vi "Format VI Info Column.vi"(8 "error in (no error)":errorcluster {"code" format="Error %.0f"}, 9 "Column":T9=enum."FP", 10 "VI Info":T1, 11 "VIDoc Printer - Confluence In":refnum<class "VIDoc Printer - Confluence.lvclass">) -> (0 "error out":errorcluster {"code" format="Error %.0f"}, 1 "Header":string, 2 "Cell Text":string, 3 "VIDoc Printer - Confluence Out":refnum<class "VIDoc Printer - Confluence.lvclass">, 4 "Viable Value?":bool, 5 "Pixel Width":i16=275)   [LabVIEW 2023, in "VIDoc Printer - Confluence.lvlib" / "VIDoc Printer - Confluence.lvclass"]
uses:
  VIDoc Printer - Confluence.lvclass
  C:/Program Files/National Instruments/LabVIEW 2023/vi.lib/DMC/VIDoc/Framework/Printer/VIDoc Printer.lvclass
  Confluence Printer Settings/VI Info Column.ctl
  <vilib>/DMC/VIDoc/Framework/Parsing/TypeDefs/Method Spec Cluster.ctl
  <vilib>/DMC/VIDoc/Framework/Parsing/TypeDefs/VI Type Extended Enum.ctl
  <vilib>/picture/picture.llb/imagedata.ctl
  <vilib>/DMC/VIDoc/Framework/Parsing/TypeDefs/Class Dispatch Type Enum.ctl
  <vilib>/DMC/VIDoc/Framework/Parsing/TypeDefs/Controls Info Cluster.ctl
  <vilib>/Utility/miscctls.llb/LVKeyTypeDef.ctl
  <vilib>/Utility/miscctls.llb/LVPointTypeDef.ctl
  <vilib>/DMC/VIDoc/Framework/Parsing/SubVIs/Structure Reporter/Tree Cluster.ctl
  Types/VI Info Image Types.ctl
  <vilib>/DMC/VIDoc/Framework/Printer/VIDoc Printer.lvclass/VIDoc Printer.ctl
  <vilib>/DMC/VIDoc/Framework/Printer/Accessors/Get Formatting Settings - Bookmark Options.vi
  <vilib>/DMC/VIDoc/Framework/Printer/Accessors/Get Formatting Settings.vi
  Accessors/Get Current Page Title.vi
  <userlib>/_PetranWay/LabVIEW Confluence API/Source/Confluence/HTML/Add Link to Text/Add URL to Text.vi
  VIDoc Printer - Confluence.lvclass/VIDoc Printer - Confluence.ctl
  <vilib>/DMC/VIDoc/Framework/Printer/VIDoc Printer.lvclass
  Confluence Formatting/Confluence Formatting.lvlib
  <userlib>/_PetranWay/LabVIEW Confluence API/Source/PetranWay_Confluence API.lvlib
  Confluence Printer Settings/VIDoc Settings - Confluence.lvclass
  <vilib>/DMC/VIDoc/Framework/Parsing/VIDoc Parsing.lvlib
  <vilib>/DMC/VIDoc/Framework/Parsing/SubVIs/Structure Reporter/Structure Reporter.lvlib
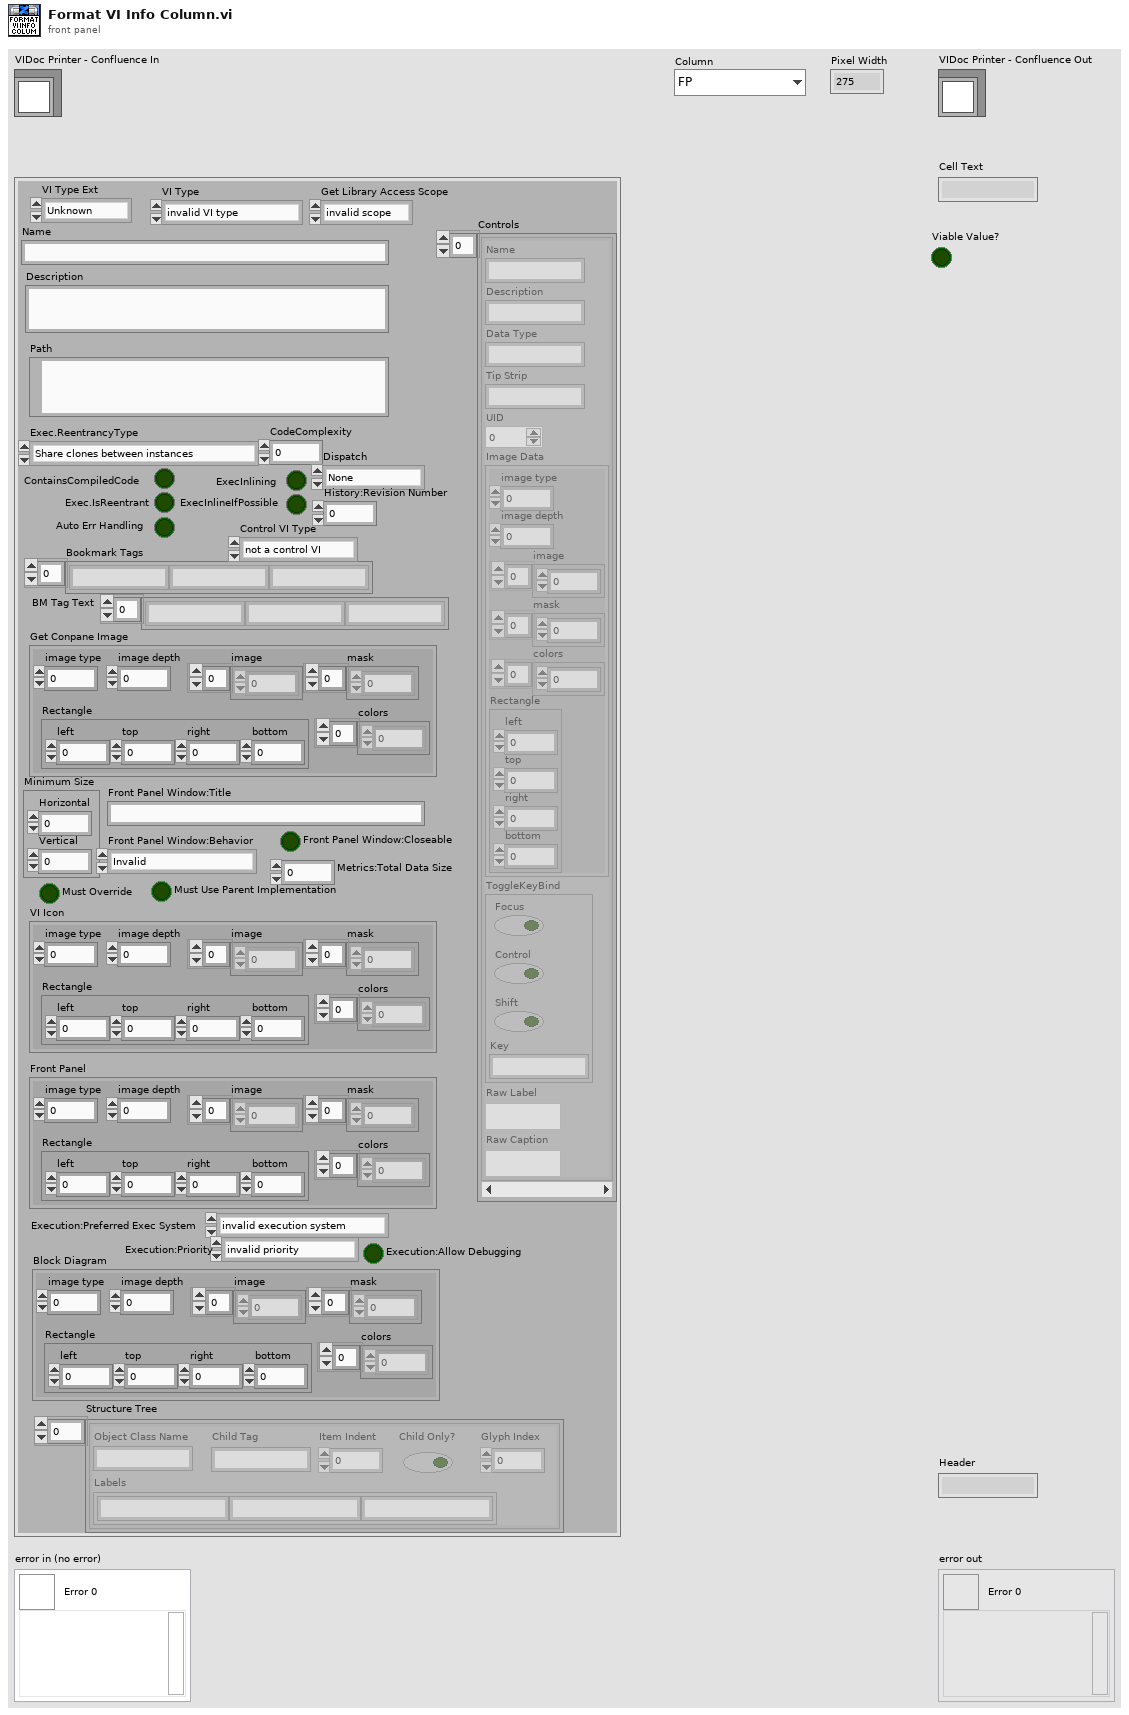
[diagram p1: front panel]
types:
  T1 = typedef "VIDoc Parsing.lvlib/Method Spec Cluster.ctl" = cluster{"VI Type Ext":T2, "Name":string, "Path":path, "Get Conpane Image":T3, "Description":string, "Get Library Access Scope":enum32{"invalid scope", "public", "private", "protected", "community"}, "Dispatch":T4, "ContainsCompiledCode":bool, "Exec.IsReentrant":bool, "Exec.ReentrancyType":enum16{"Share clones between instances", "Preallocate clone for each instance"}, "ExecInlining":bool, "ExecInlineIfPossible":bool, "Auto Err Handling":bool, "CodeComplexity":sgl, "Bookmark Tags":string[], "Control VI Type":enum32{"not a control VI", "control", "typedef", "strict typedef"}, "Controls":T5[], "VI Type":enum32{"invalid VI type", "Standard VI", "Control VI", "Global VI", "Polymorphic VI", "Configuration VI", "SubSystem", "Facade VI", "Method VI", "Statechart Diagram VI"}, "Minimum Size":T7, "Front Panel Window:Title":string, "Front Panel Window:Behavior":enum32{"Invalid", "Default", "Floating", "Floating/Auto-Hide", "Modal"}, "Front Panel Window:Closeable":bool, "Must Override":bool, "Must Use Parent Implementation":bool, "VI Icon":T3, "Front Panel":T3, "History:Revision Number":u32, "Metrics:Total Data Size":u32, "Execution:Allow Debugging":bool, "Execution:Preferred Exec System":enum32{"invalid execution system", "user interface", "standard", "instrument i/o", "data acquisition", "other 1", "other 2", "same as caller"}, "Execution:Priority":enum32{"invalid priority", "background priority", "normal priority", "above normal priority", "high priority", "time critical priority", "subroutine"}, "BM Tag Text":string[], "Block Diagram":T3, "Structure Tree":T8[]}
  T2 = typedef "VIDoc Parsing.lvlib/VI Type Extended Enum.ctl" = enum16{"Unknown", "Class Method", "Class Accessor Get", "Class Accessor Set", "Class Control", "Library Method", "Library Control", "VI", "Control"}
  T3 = typedef "imagedata.ctl" = cluster{"image type":i32, "image depth":i32, "image":u8[], "mask":u8[], "colors":u32[], "Rectangle":cluster{"left":i16, "top":i16, "right":i16, "bottom":i16}}
  T4 = typedef "VIDoc Parsing.lvlib/Class Dispatch Type Enum.ctl" = enum16{"None", "Static", "Dynamic"}
  T5 = typedef "VIDoc Parsing.lvlib/Controls Info Cluster.ctl" = cluster{"Name":string, "Description":string, "Data Type":string, "Tip Strip":string, "UID":i32, "Image Data":T3, "ToggleKeyBind":T6, "Raw Label":string, "Raw Caption":string}
  T6 = typedef "LVKeyTypeDef.ctl" = cluster{"Focus":bool, "Control":bool, "Shift":bool, "Key":string}
  T7 = typedef "LVPointTypeDef.ctl" = cluster{"Horizontal":i16, "Vertical":i16}
  T8 = typedef "VIDoc Parsing.lvlib/Structure Reporter.lvlib/Tree Cluster.ctl" = cluster{"Object Class Name":string, "Labels":string[], "Child Tag":string, "Item Indent":i32, "Child Only?":bool, "Glyph Index":i32}
  T9 = typedef "VIDoc Printer - Confluence.lvlib/VIDoc Settings - Confluence.lvclass/VI Info Column.ctl" = enum16{"Name", "Conpane", "BD", "FP", "VI Icon", "Description", "Reentrant", "Inline", "Auto Error", "Compiled", "Code Complexity", "Data Size", "Debug", "Priority", "Rev", "Minimum Size", "Title", "FP Behavior", "FP Closeable", "Author", "Commit Hash", "Last Change", "Branch", "Scope", "Type", "Dispatch", "Must Override", "Must Use Parent", "Structure Tree"}
  T10 = typedef "VIDoc Printer - Confluence.lvlib/VIDoc Printer - Confluence.lvclass/VI Info Image Types.ctl" = enum16{"Conpane", "FP", "BD", "Icon"}
  T11 = typedef "VIDoc Printer.lvlib/Printer Settings.lvclass/Bookmark Options.ctl" = cluster{"Bookmarks as New Line in VI Descriptions":bool, "Unique Bookmark Tags Only":bool, "Include Tag and Text":bool}
  T12 = enum16{"Share clones between instances", "Preallocate clone for each instance"}
  T13 = typedef "VIDoc Printer.lvlib/Printer Settings.lvclass/Formatting Options.ctl" = cluster{"Background":cluster{"Public Scope":T14, "Protected Scope":T14, "Community Scope":T14, "Private Scope":T14, "Unknown Scope":T14, "Auto Error Handling":T14, "Inline":T14, "Separate CC":T14, "Execution Priority Normal":T14, "Reentrancy Non-RE":T14}, "Bookmark Options":T11}
  T14 = typedef "VIDoc Printer.lvlib/Printer Settings.lvclass/Background Formatting Cluster.ctl" = cluster{"Option":bool, "Color":u32, "Operator":bool}
  T15 = enum32{"invalid priority", "background priority", "normal priority", "above normal priority", "high priority", "time critical priority", "subroutine"}
  T16 = enum32{"Invalid", "Default", "Floating", "Floating/Auto-Hide", "Modal"}
  T17 = cluster{"Timestamp":timestamp, "Commit Hash":string, "Author Name":string, "Branch":string, "Commit Hash URL":string}
  T18 = enum32{"invalid scope", "public", "private", "protected", "community"}
  T19 = enum32{"not a control VI", "control", "typedef", "strict typedef"}
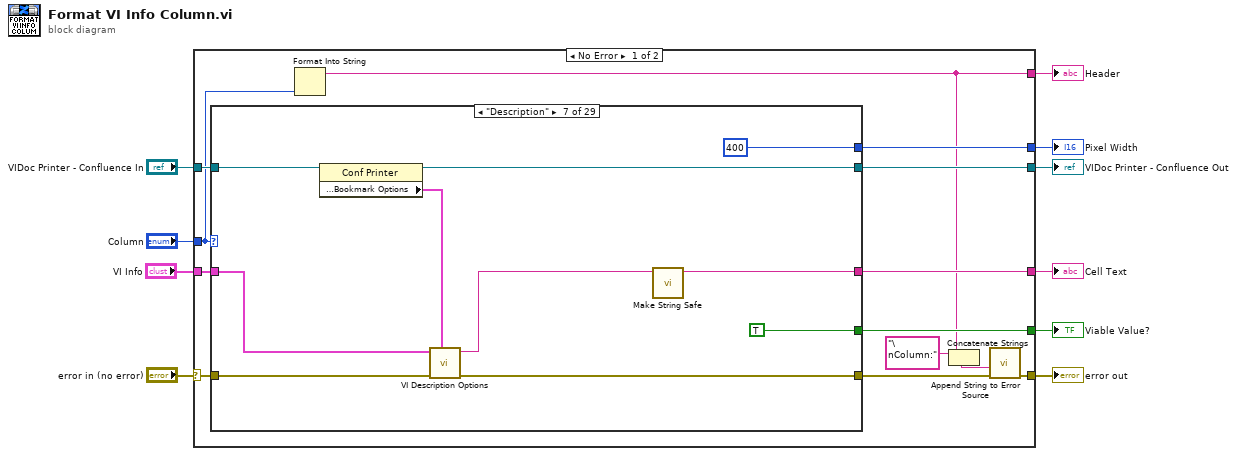
[diagram p0: block diagram]
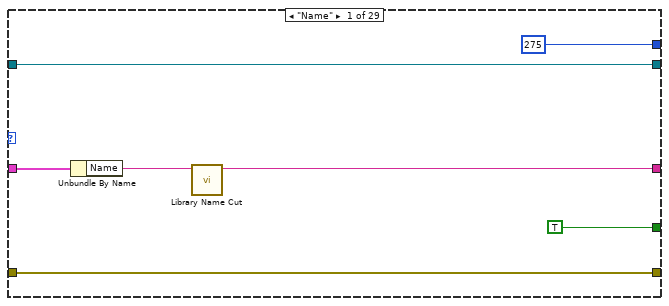
[diagram p2: hidden frame]
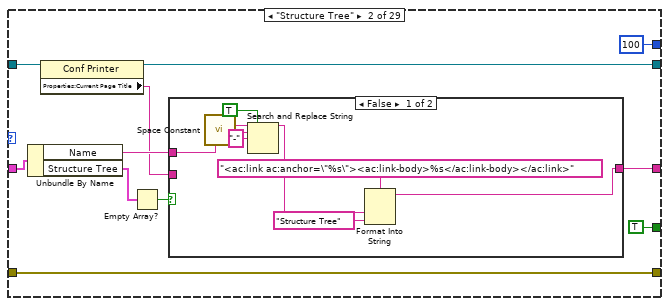
[diagram p3: hidden frame]
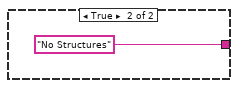
[diagram p4: hidden frame]
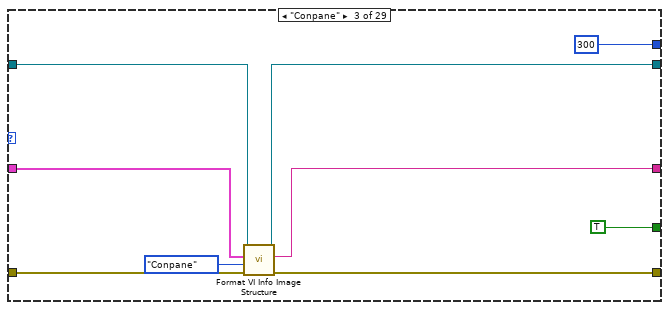
[diagram p5: hidden frame]
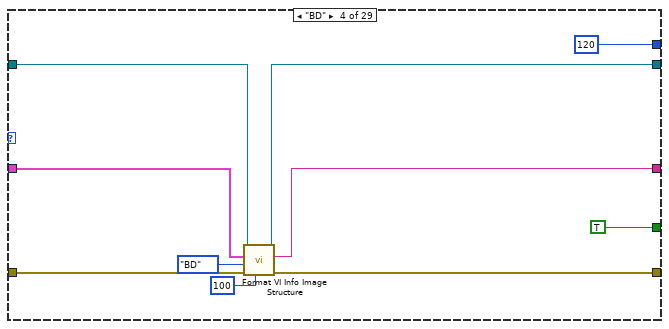
[diagram p6: hidden frame]
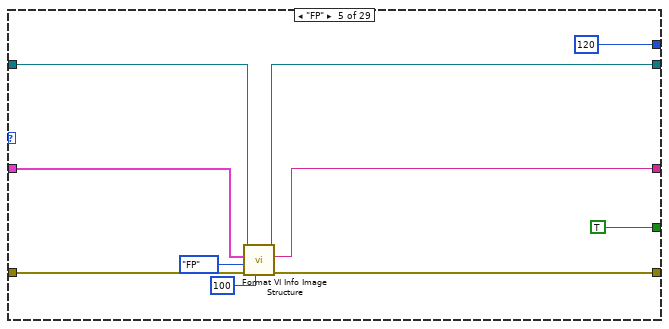
[diagram p7: hidden frame]
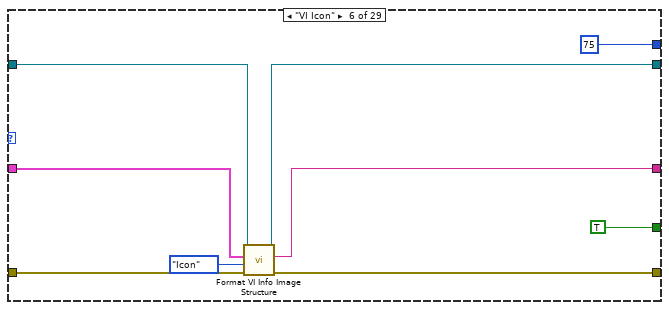
[diagram p8: hidden frame]
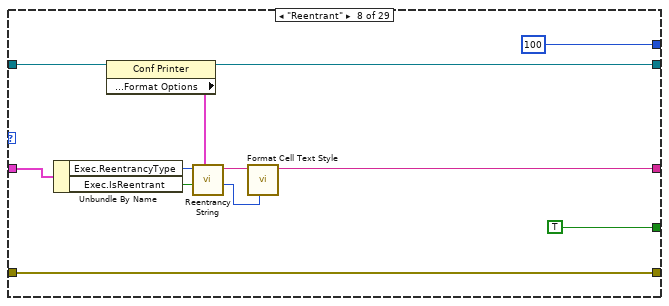
[diagram p9: hidden frame]
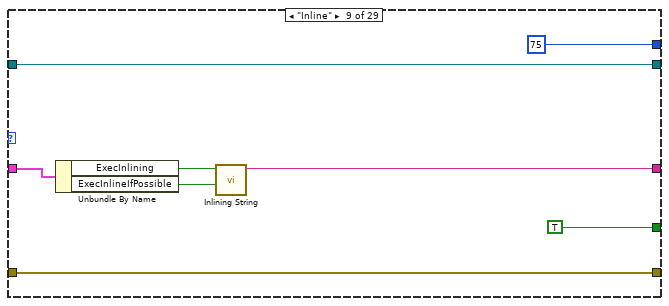
[diagram p10: hidden frame]
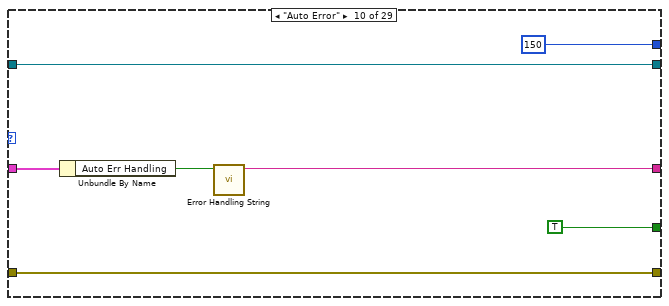
[diagram p11: hidden frame]
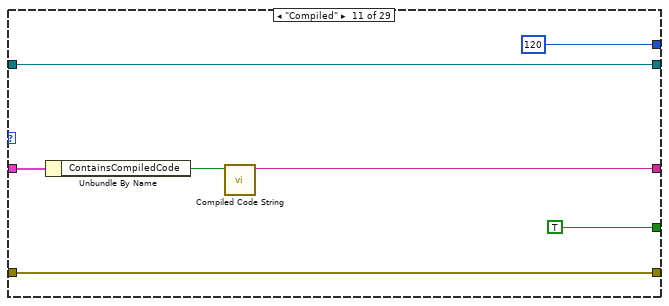
[diagram p12: hidden frame]
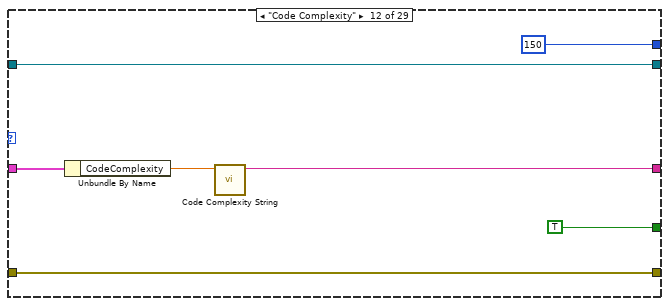
[diagram p13: hidden frame]
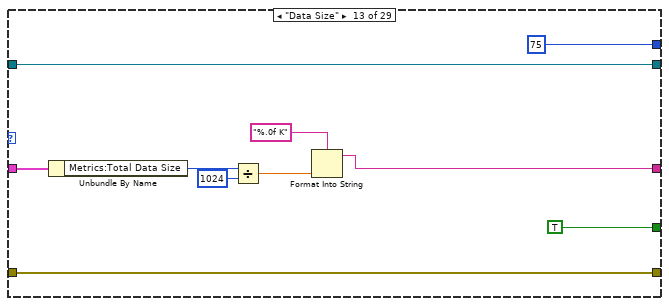
[diagram p14: hidden frame]
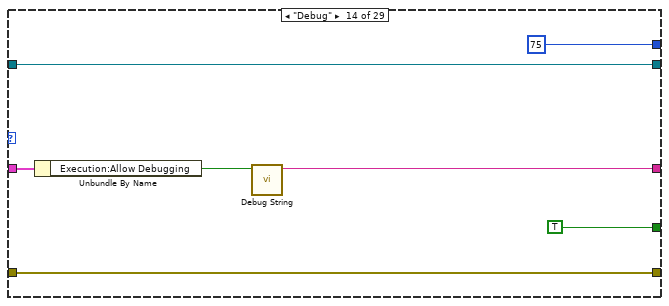
[diagram p15: hidden frame]
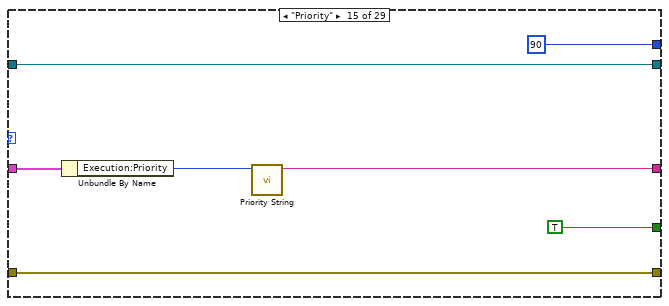
[diagram p16: hidden frame]
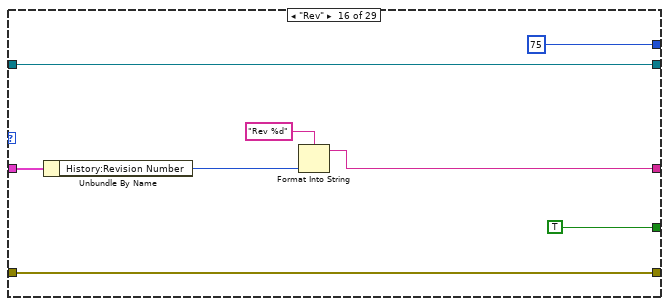
[diagram p17: hidden frame]
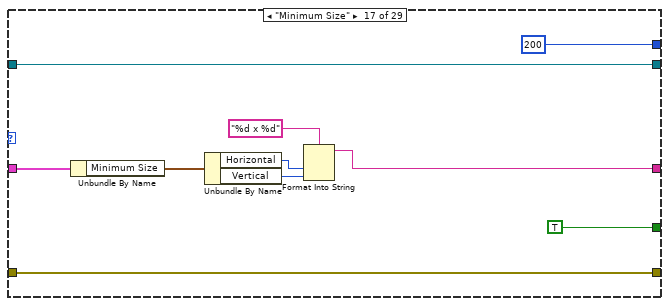
[diagram p18: hidden frame]
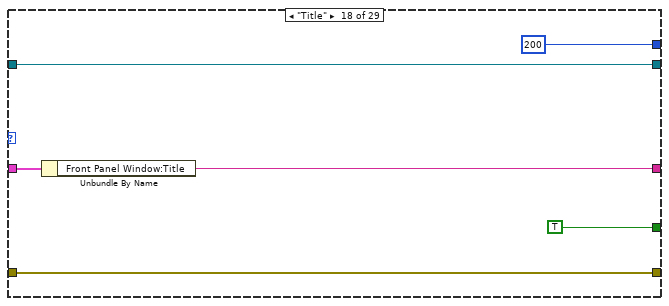
[diagram p19: hidden frame]
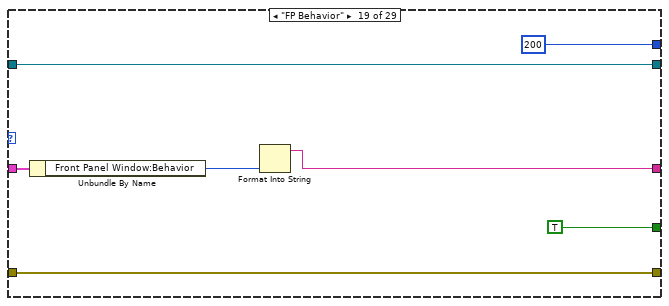
[diagram p20: hidden frame]
diagram:
  n1 = case shown="No Error" "error in (no error)" {
    selector: "error in (no error)" -> [w22 w293]
    tunnel: [w14 w293] -> w9
    tunnel: [w21 w292] -> w7
    tunnel: "VIDoc Printer - Confluence In" -> [w20 w292]
    tunnel: "Column" -> [w17 _]
    tunnel: "VI Info" -> [w19 _]
    tunnel: [w18 _] -> w4
    tunnel: [w12 _] -> w3
    tunnel: [w16 _] -> w2
    tunnel: [w15 FALSE ("File Change Info Available?")] -> w1
    frame No Error {
      n2 = case shown="\"Description\"" w17 {
        tunnel: [w30 w40 w55 w65 w75 w84 w91 w104 w115 w122 w129 w136 w146 w153 w160 w168 w178 w184 w191 w200 w211 w214 w243 w253 w262 w269 w273 w280 w287] -> w23
        tunnel: w22 -> [w30 w40 w58 w68 w78 w87 w96 w104 w115 w122 w129 w136 w146 w153 w160 w168 w178 w184 w191 w200 w210 w224 w242 w252 w262 w269 w273 w280 w287]
        tunnel: [w29 w32 w56 w66 w76 w85 w95 w108 w117 w124 w131 w138 w148 w155 w162 w170 w180 w186 w193 w202 w209 w223 w241 w251 w261 w268 w275 w282 w289] -> w21
        tunnel: w20 -> [w29 w41 w57 w67 w77 w86 w97 w109 w117 w124 w131 w138 w148 w155 w162 w170 w180 w186 w193 w202 w208 w222 w240 w250 w261 w268 w275 w282 w289]
        tunnel: w19 -> [w28 w39 w52 w62 w72 w81 w93 w107 w116 w123 w130 w137 w147 w154 w161 w169 w179 w185 w192 w201 w212 w225 w244 w254 w260 w267 w274 w281 w288]
        tunnel: [w25 w35 w54 w64 w74 w83 w89 w100 w112 w120 w127 w134 w141 w151 w158 w165 w173 w183 w189 w196 w205 w215 w235 w247 w256 w263 w270 w277 w284] -> w18
        tunnel: [i16 275 ("Pixel Width") i16 100 ("Pixel Width") i16 300 ("Pixel Width") i16 120 ("Pixel Width") i16 120 ("Pixel Width") i16 75 ("Pixel Width") i16 400 ("Pixel Width") i16 100 ("Pixel Width") i16 75 ("Pixel Width") i16 150 ("Pixel Width") i16 120 ("Pixel Width") i16 150 ("Pixel Width") i16 75 ("Pixel Width") i16 75 ("Pixel Width") i16 90 ("Pixel Width") i16 75 ("Pixel Width") i16 200 ("Pixel Width") i16 200 ("Pixel Width") i16 200 ("Pixel Width") i16 120 ("Pixel Width") i16 120 ("Pixel Width") i16 120 ("Pixel Width") i16 200 ("Pixel Width") i16 200 ("Pixel Width") i16 100 ("Pixel Width") i16 300 ("Pixel Width") i16 90 ("Pixel Width") i16 90 ("Pixel Width") i16 90 ("Pixel Width")] -> w16
        tunnel: [TRUE ("File Change Info Available?") TRUE ("File Change Info Available?") TRUE ("File Change Info Available?") TRUE ("File Change Info Available?") TRUE ("File Change Info Available?") TRUE ("File Change Info Available?") TRUE ("File Change Info Available?") TRUE ("File Change Info Available?") TRUE ("File Change Info Available?") TRUE ("File Change Info Available?") TRUE ("File Change Info Available?") TRUE ("File Change Info Available?") TRUE ("File Change Info Available?") TRUE ("File Change Info Available?") TRUE ("File Change Info Available?") TRUE ("File Change Info Available?") TRUE ("File Change Info Available?") TRUE ("File Change Info Available?") TRUE ("File Change Info Available?") TRUE ("File Change Info Available?") TRUE ("File Change Info Available?") w220 w234 w246 TRUE ("File Change Info Available?") TRUE ("File Change Info Available?") TRUE ("File Change Info Available?") TRUE ("File Change Info Available?") TRUE ("File Change Info Available?")] -> w15
        frame "Name" {
          n3 = Unbundle By Name(w28) -> ("Name"=w27:string)
          n4 = call "Library Name Cut.vi"("Name in"=w27) -> ("Name out"=w25:string)  [unwired: 10 in]
        }
        frame "Structure Tree" {
          n5 = Unbundle By Name(w39) -> ("Name"=w33:string, "Structure Tree"=w34:T8[])
          n6 = property class="Conf Printer"(reference=w41) -> (reference out=w32:refnum<class "VIDoc Printer - Confluence.lvclass">, "Properties:Current Page Title"=w31:string)  [unwired: 1 in, 1 out]
          n7 = Empty Array?(array=w34) -> (empty?=w36:bool)
          n8 = case shown="False" w36 {
            tunnel: [w43 "No Structures"] -> w35
            tunnel: w33 -> [w47 _]
            tunnel: w31 -> [_ _]
            frame False {
              n9 = call <vilib>:"Space Constant.vi"() -> ("String"=w49:string)
              n10 = Search and Replace String(replace all?=TRUE ("replace all? (F)"), input string=w47, search string=w49, replace string="-" ("replace string (\"\")")) -> (result string=w45:string)  [unwired: 4 in, 3 out]
              n11 = Format Into String(format string="<ac:link ac:anchor=\"%s\"><ac:link-body>%s</ac:link-body></ac:link>", w45, "Structure Tree" ("input 2")) -> (resulting string=w43:string)  [unwired: 2 in, 1 out]
            }
            frame True {
            }
          }
        }
        frame "Conpane" {
          n12 = call "Format VI Info Image Structure.vi"("Error in"=w58, "Image Type"=VI_Info_Image_Types."Conpane", "VI Info"=w52, "VIDoc Printer - Confluence In"=w57) -> ("Error out"=w55:errorcluster, "Image Structure Text"=w54:string, "VIDoc Printer - Confluence Out"=w56:refnum<class "VIDoc Printer - Confluence.lvclass">)  [unwired: 4 in, 1 out]
        }
        frame "BD" {
          n13 = call "Format VI Info Image Structure.vi"("Max Width (500 pixels)"=i16 100, "Error in"=w68, "Image Type"=VI_Info_Image_Types."BD", "VI Info"=w62, "VIDoc Printer - Confluence In"=w67) -> ("Error out"=w65:errorcluster, "Image Structure Text"=w64:string, "VIDoc Printer - Confluence Out"=w66:refnum<class "VIDoc Printer - Confluence.lvclass">)  [unwired: 3 in, 1 out]
        }
        frame "FP" {
          n14 = call "Format VI Info Image Structure.vi"("Max Width (500 pixels)"=i16 100, "Error in"=w78, "Image Type"=VI_Info_Image_Types."FP", "VI Info"=w72, "VIDoc Printer - Confluence In"=w77) -> ("Error out"=w75:errorcluster, "Image Structure Text"=w74:string, "VIDoc Printer - Confluence Out"=w76:refnum<class "VIDoc Printer - Confluence.lvclass">)  [unwired: 3 in, 1 out]
        }
        frame "VI Icon" {
          n15 = call "Format VI Info Image Structure.vi"("Error in"=w87, "Image Type"=VI_Info_Image_Types."Icon", "VI Info"=w81, "VIDoc Printer - Confluence In"=w86) -> ("Error out"=w84:errorcluster, "Image Structure Text"=w83:string, "VIDoc Printer - Confluence Out"=w85:refnum<class "VIDoc Printer - Confluence.lvclass">)  [unwired: 4 in, 1 out]
        }
        frame "Description" {
          n16 = property class="Conf Printer"(reference=w97) -> (reference out=w95:refnum<class "VIDoc Printer - Confluence.lvclass">, "Properties:Settings:Formatting Options:Bookmark Options"=w94:T11)  [unwired: 1 in, 1 out]
          n17 = call <vilib>:"VI Description Options.vi"("Bookmark Options"=w94, "Error in"=w96, "VI Info"=w93) -> ("Error out"=w91:errorcluster, "Description"=w92:string)  [unwired: 7 in]
          n18 = call "Make String Safe.vi"("Raw String"=w92) -> ("String out"=w89:string)  [unwired: 9 in, 1 out]
        }
        frame "Reentrant" {
          n19 = Unbundle By Name(w107) -> ("Exec.ReentrancyType"=w106:T12, "Exec.IsReentrant"=w105:bool)
          n20 = property class="Conf Printer"(reference=w109) -> (reference out=w108:refnum<class "VIDoc Printer - Confluence.lvclass">, "Properties:Settings:Formatting Options:Format Options"=w101:T13)  [unwired: 1 in, 1 out]
          n21 = call <vilib>:"Reentrancy String.vi"("Format Options"=w101, "Exec.IsReentrant"=w105, "Exec.ReentrancyType"=w106) -> ("Cell Color"=w102:u32, "Reentrancy"=w103:string)  [unwired: 7 in]
          n22 = call "Format Cell Text Style.vi"("BG Color (Unchanged)"=w102, "String"=w103) -> ("Formatted Text"=w100:string)  [unwired: 8 in, 1 out]
        }
        frame "Inline" {
          n23 = Unbundle By Name(w116) -> ("ExecInlining"=w114:bool, "ExecInlineIfPossible"=w113:bool)
          n24 = call <vilib>:"Inlining String.vi"("ExecInlineIfPossible"=w113, "ExecInlining"=w114) -> ("Inline Text"=w112:string)  [unwired: 9 in]
        }
        frame "Auto Error" {
          n25 = Unbundle By Name(w123) -> ("Auto Err Handling"=w121:bool)
          n26 = call <vilib>:"Error Handling String.vi"("Auto Err Handling"=w121) -> ("Error Handling String"=w120:string)  [unwired: 10 in]
        }
        frame "Compiled" {
          n27 = Unbundle By Name(w130) -> ("ContainsCompiledCode"=w128:bool)
          n28 = call <vilib>:"Compiled Code String.vi"("ContainsCompiledCode"=w128) -> ("Compiled Code String"=w127:string)  [unwired: 10 in]
        }
        frame "Code Complexity" {
          n29 = Unbundle By Name(w137) -> ("CodeComplexity"=w135:sgl)
          n30 = call <vilib>:"Code Complexity String.vi"("CodeComplexity"=w135) -> ("Code Complexity String"=w134:string)  [unwired: 10 in]
        }
        frame "Data Size" {
          n31 = Unbundle By Name(w147) -> ("Metrics:Total Data Size"=w142:u32)
          n32 = Divide(x=w142, y=u32 1024) -> (x/y=w143:dbl)
          n33 = Format Into String(format string="%.0f K", w143) -> (resulting string=w141:string)  [unwired: 2 in, 1 out]
        }
        frame "Debug" {
          n34 = Unbundle By Name(w154) -> ("Execution:Allow Debugging"=w152:bool)
          n35 = call <vilib>:"Debug String.vi"("Allow Debugging"=w152) -> ("Debug String"=w151:string)  [unwired: 10 in]
        }
        frame "Priority" {
          n36 = Unbundle By Name(w161) -> ("Execution:Priority"=w159:T15)
          n37 = call <vilib>:"Priority String.vi"("Execution:Priority"=w159) -> ("Priority String"=w158:string)  [unwired: 10 in]
        }
        frame "Rev" {
          n38 = Unbundle By Name(w169) -> ("History:Revision Number"=w166:u32)
          n39 = Format Into String(format string="Rev %d", w166) -> (resulting string=w165:string)  [unwired: 2 in, 1 out]
        }
        frame "Minimum Size" {
          n40 = Unbundle By Name(w179) -> ("Minimum Size"=w174:T7)
          n41 = Unbundle By Name(w174) -> ("Horizontal"=w177:i16, "Vertical"=w176:i16)
          n42 = Format Into String(format string="%d x %d", w177, w176) -> (resulting string=w173:string)  [unwired: 2 in, 1 out]
        }
        frame "Title" {
          n43 = Unbundle By Name(w185) -> ("Front Panel Window:Title"=w183:string)
        }
        frame "FP Behavior" {
          n44 = Unbundle By Name(w192) -> ("Front Panel Window:Behavior"=w190:T16)
          n45 = Format Into String(w190) -> (resulting string=w189:string)  [unwired: 3 in, 1 out]
        }
        frame "FP Closeable" {
          n46 = Unbundle By Name(w201) -> ("Front Panel Window:Closeable"=w199:bool)
          n47 = Select(t="Closable" ("format string"), s=w199, f="Not Closable" ("format string")) -> (s? t:f=w196:string)
        }
        frame "Author" {
          n48 = Unbundle By Name(w212) -> ("Path"=w207:path)
          n49 = call "Retrieve File Change Info.vi"("error in (no error)"=w210, "Absolute File Path"=w207, "VIDoc Printer - Confluence In"=w208) -> ("error out"=w211:errorcluster, "File Change Info"=w206:T17, "VIDoc Printer - Confluence Out"=w209:refnum<class "VIDoc Printer - Confluence.lvclass">)  [unwired: 5 in, 1 out]
          n50 = Unbundle By Name(w206) -> ("Author Name"=w205:string)
        }
        frame "Commit Hash" {
          n51 = Unbundle By Name(w225) -> ("Path"=w221:path)
          n52 = call "Retrieve File Change Info.vi"("error in (no error)"=w224, "Absolute File Path"=w221, "VIDoc Printer - Confluence In"=w222) -> ("error out"=w217:errorcluster, "File Change Info Available?"=w220:bool, "File Change Info"=w216:T17, "VIDoc Printer - Confluence Out"=w223:refnum<class "VIDoc Printer - Confluence.lvclass">)  [unwired: 5 in]
          n53 = Unbundle By Name(w216) -> ("Commit Hash"=w219:string, "Commit Hash URL"=w218:string)
          n54 = case shown="\"\"" w218 {
            selector: w218 -> [_ w231]
            tunnel: w219 -> [w228 w233]
            tunnel: [w228 w232] -> w215
            tunnel: w217 -> [w227 w230]
            tunnel: [w227 w229] -> w214
            frame "" {
            }
            frame Default {
              n55 = call-poly <userlib>:"Add Link to Text.vi"("Text"=w233, "URL"=w231, "error in (no error)"=w230) -> ("HTML Text String"=w232:string, "error out"=w229:errorcluster)  [unwired: 10 in, 1 out]
            }
          }
        }
        frame "Last Change" {
          n56 = Unbundle By Name(w244) -> ("Path"=w239:path)
          n57 = call "Retrieve File Change Info.vi"("error in (no error)"=w242, "Absolute File Path"=w239, "VIDoc Printer - Confluence In"=w240) -> ("error out"=w243:errorcluster, "File Change Info Available?"=w234:bool, "File Change Info"=w238:T17, "VIDoc Printer - Confluence Out"=w241:refnum<class "VIDoc Printer - Confluence.lvclass">)  [unwired: 5 in]
          n58 = Unbundle By Name(w238) -> ("Timestamp"=w237:timestamp)
          n59 = Format Into String(format string="%<%Y/%m/%d %H:%M:%S>T", w237) -> (resulting string=w235:string)  [unwired: 2 in, 1 out]
        }
        frame "Branch" {
          n60 = Unbundle By Name(w254) -> ("Path"=w249:path)
          n61 = call "Retrieve File Change Info.vi"("error in (no error)"=w252, "Absolute File Path"=w249, "VIDoc Printer - Confluence In"=w250) -> ("error out"=w253:errorcluster, "File Change Info Available?"=w246:bool, "File Change Info"=w248:T17, "VIDoc Printer - Confluence Out"=w251:refnum<class "VIDoc Printer - Confluence.lvclass">)  [unwired: 5 in]
          n62 = Unbundle By Name(w248) -> ("Branch"=w247:string)
        }
        frame "Scope" {
          n63 = Unbundle By Name(w260) -> ("Get Library Access Scope"=w257:T18)
          n64 = call <vilib>:"Scope String.vi"("Get Library Access Scope"=w257) -> ("String"=w256:string)  [unwired: 10 in]
        }
        frame "Type" {
          n65 = Unbundle By Name(w267) -> ("Control VI Type"=w264:T19)
          n66 = call <vilib>:"Control Type to String.vi"("Control VI Type"=w264) -> ("String"=w263:string)  [unwired: 10 in]
        }
        frame "Dispatch" {
          n67 = Unbundle By Name(w274) -> ("Dispatch"=w271:T4)
          n68 = Format Into String(w271) -> (resulting string=w270:string)  [unwired: 3 in, 1 out]
        }
        frame "Must Override" {
          n69 = Unbundle By Name(w281) -> ("Must Override"=w278:bool)
          n70 = Format Into String(w278) -> (resulting string=w277:string)  [unwired: 3 in, 1 out]
        }
        frame "Must Use Parent" {
          n71 = Unbundle By Name(w288) -> ("Must Use Parent Implementation"=w285:bool)
          n72 = Format Into String(w285) -> (resulting string=w284:string)  [unwired: 3 in, 1 out]
        }
      }
      n73 = Format Into String(w17) -> (resulting string=w12:string)  [unwired: 3 in, 1 out]
      n74 = Concatenate Strings("\nColumn:" ("string"), w12) -> (w11:string)
      n75 = call "Append String to Error Source.vi"("Error In"=w23, "String to Append"=w11) -> ("Error Out"=w14:errorcluster)  [unwired: 9 in]
    }
    frame Error {
    }
  }
  "error out" <- w9
  "VIDoc Printer - Confluence Out" <- w7
  "Pixel Width" <- w2
  "Cell Text" <- w4
  "Header" <- w3
  "Viable Value?" <- w1
